vi "Cascade State.vi"(6 "First Iteration?":bool, 10 "Positions":T3, 11 "Cascade Motors":T1) -> (3 "Is Finished?":bool=TRUE)   [LabVIEW 2023]
uses:
  <vilib>/REV Custom Controls/Spark Output Control Type.ctl
  <vilib>/REVLibDriver/REVLibDriver.lvlib
  <resource>/objmgr/REVSpark.rc
  <vilib>/MRC/MrcLib.lvlib
  <vilib>/REV Custom Controls/SPARK Closed Loop Slot.ctl
  Cascade Positions.ctl
  <vilib>/REV Custom Controls/REVSparkRefnum.ctl
panel:
  in  "Cheat Factor":dbl=10.0
  out "Velocity":T2(graph)
  in  "dP":dbl
  out "Distance":dbl=-0.5875421712011715
  in  "Velocity Max":dbl=9000.0
  in  "Acceleration Max":dbl=9000.0
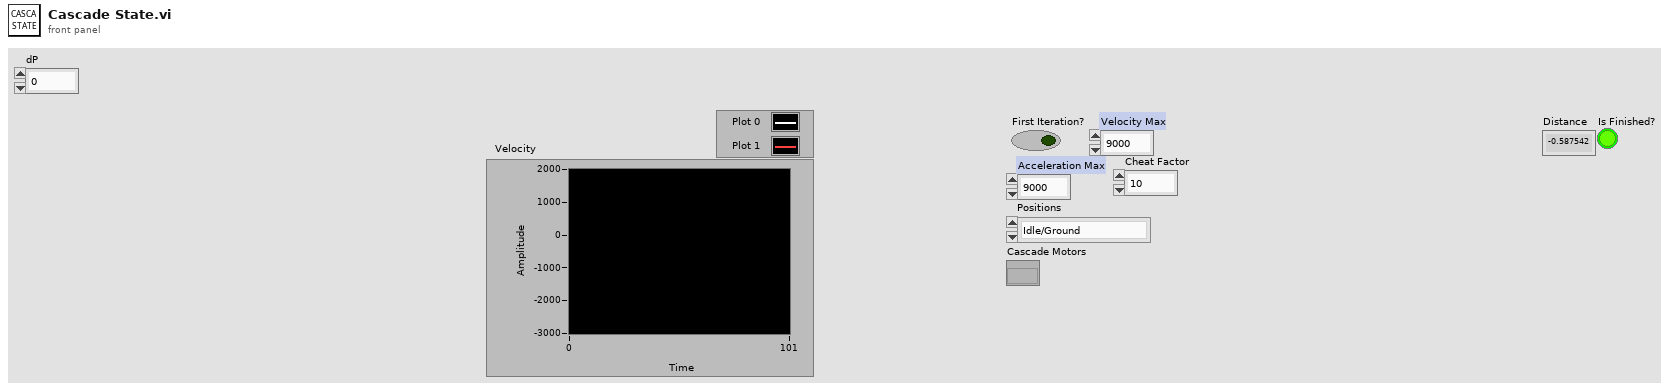
[diagram p1: front panel]
types:
  T1 = typedef "REVLibDriver.lvlib/REVSparkRefnum.ctl" = refnum<k20>
  T2 = cluster{"Numeric":dbl, "EncoderVelocityValue":sgl}
  T3 = typedef "Cascade Positions.ctl" = enum16{"Idle/Ground", "Raised L1", "L2", "L2 Tip", "L3", "L3 Tip", "Feeder", "\"Default\""}
  T4 = cluster{"Array":cluster{"Preset Name":T3, "Cascade Pos":dbl}[]}
  T5 = typedef "REVLibDriver.lvlib/Spark Output Control Type.ctl" = enum16{"Percent VBus", "Velocity", "Voltage", "Position", "Current", "MAXMotion Position", "MAXMotion Velocity"}
  T6 = typedef "SPARK Closed Loop Slot.ctl" = u16
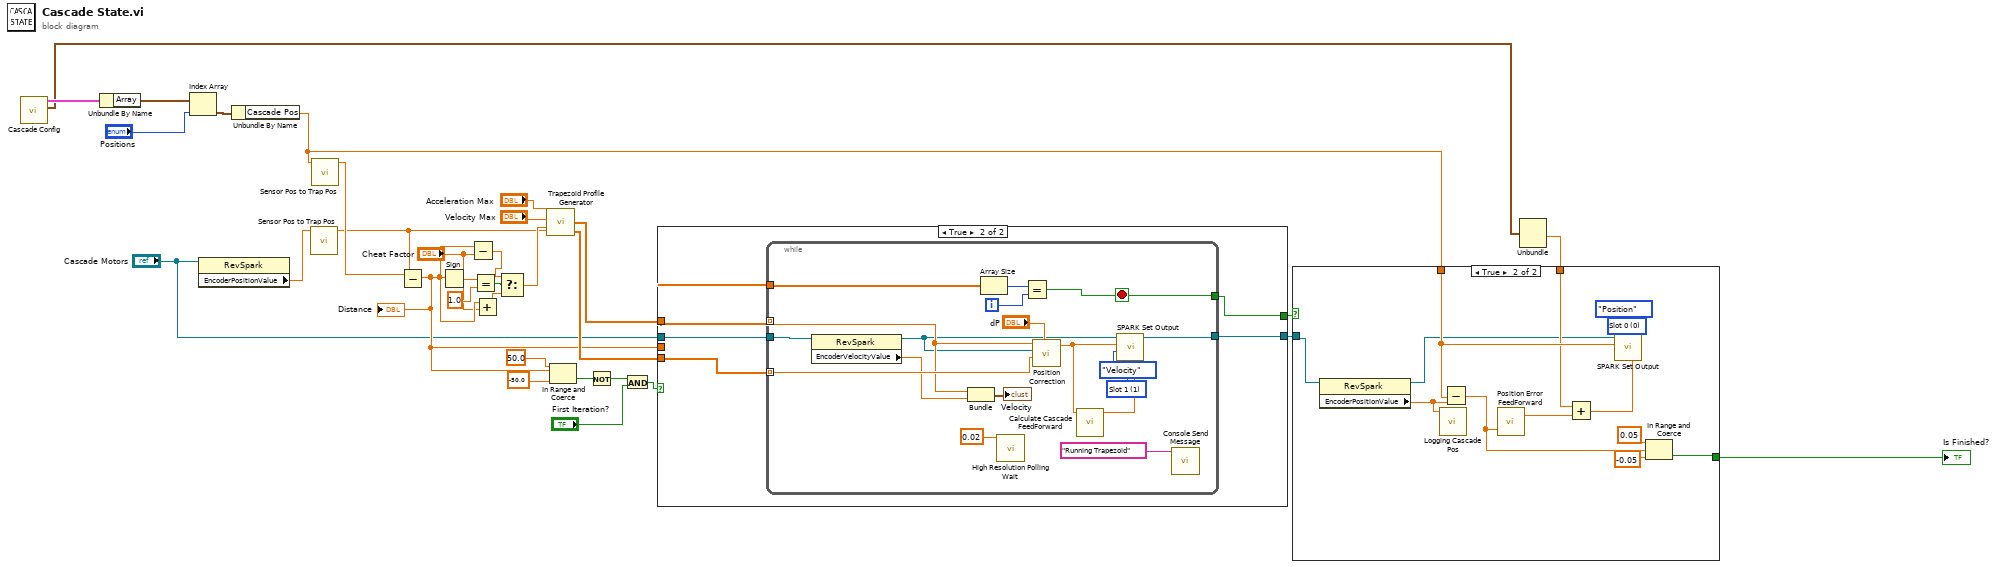
[diagram p0: block diagram]
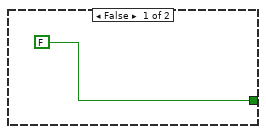
[diagram p2: hidden frame]
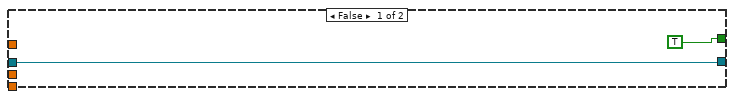
[diagram p3: hidden frame]
diagram:
  n1 = call "Cascade Config.vi"() -> ("FeedForward Constants Out"=w16:cluster{"kA":dbl, "kS":dbl, "kG":dbl, "kV":dbl}, "Cascade Setpoints Config Out (Sensor Positions)"=w32:T4)  [unwired: 10 in]
  n2 = Unbundle By Name(w32) -> ("Array"=w31:cluster{"Preset Name":T3, "Cascade Pos":dbl}[])
  n3 = Index Array(array=w31, index="Positions") -> (element=w30:cluster{"Preset Name":T3, "Cascade Pos":dbl})
  n4 = property class="RevSpark"(reference="Cascade Motors") -> ("EncoderPositionValue"=w23:sgl)  [unwired: 1 in, 2 out]
  n5 = Unbundle By Name(w30) -> ("Cascade Pos"=w25:dbl)
  n6 = call "Sensor Pos to Trap Pos.vi"("Sensor Pos"=w23) -> ("Trapezoid Pos"=w2:dbl)  [unwired: 10 in]
  n7 = call "Sensor Pos to Trap Pos.vi"("Sensor Pos"=w25) -> ("Trapezoid Pos"=w24:dbl)  [unwired: 10 in]
  n8 = Subtract(x=w24, y=w2) -> (x-y=w8:dbl)
  "Distance" <- w8
  n9 = Sign(1:w8) -> (0:w13:dbl)
  n10 = Subtract(x=w8, y="Cheat Factor") -> (x-y=w10:dbl)
  n11 = Equal?(x=w13, y=1.0 ("x")) -> (x = y?=w11:bool)
  n12 = Add(x=w8, y="Cheat Factor") -> (x+y=w9:dbl)
  n13 = Select(t=w10, s=w11, f=w9) -> (s? t:f=w6:dbl)
  n14 = call "Trapezoid Profile Generator.vi"("Starting Position"=w2, "Distance"=w6, "Velocity Max"="Velocity Max", "Acceleration Max"="Acceleration Max") -> ("Positions"=w22:dbl[], "Velocity values"=w27:dbl[])  [unwired: 5 in, 1 out]
  n15 = In Range and Coerce(upper limit=50.0, x=w8, lower limit=-50.0) -> (In Range?=w19:bool)  [unwired: 1 out]
  n16 = Not(x=w19) -> (.not. x?=w17:bool)
  n17 = And(x=w17, y="First Iteration?") -> (x .and. y?=w18:bool)
  n18 = case shown="True" w18 {
    tunnel: w27 -> [_ w39]
    tunnel: "Cascade Motors" -> [w33 w38]
    tunnel: [TRUE w37] -> w4
    tunnel: [w33 w36] -> w26
    tunnel: w22 -> [_ w35]
    tunnel: w8 -> [_ _]
    frame False {
    }
    frame True {
      n19 = while {
        tunnel: w39 -> [w47] mode=indexing
        tunnel: w38 -> [w46]
        tunnel: w39 -> [w56]
        tunnel: [w48] -> w37
        tunnel: [w53] -> w36
        tunnel: w35 -> [w52] mode=indexing
        i -> [w57]
        stop <- w48 stop-if-true
        w40 = T6 1 items=["Slot 0", "Slot 1", "Slot 2", "Slot 3"] ("Closed Loop Slot")
        n20 = property class="RevSpark"(reference=w46) -> (reference out=w42:T1, "EncoderVelocityValue"=w45:sgl)  [unwired: 1 in, 1 out]
        n21 = Bundle("Numeric"=w47, "EncoderVelocityValue"=w45) -> (→"Velocity":T2)  [unwired: 1 in]
        n22 = Array Size(array=w56) -> (size(s)=w55:i32)
        n23 = call <vilib>:"High Resolution Polling Wait.vi"("seconds to wait"=0.02) -> ()  [unwired: 10 in, 1 out]
        n24 = Equal?(x=w55, y=w57) -> (x = y?=w48:bool)
        n25 = call "Position Correction.vi"("dP"="dP", "Pos In"=w52, "RevSpark Session"=w42, "Velocity In"=w47) -> ("Velocity Out"=w51:dbl)  [unwired: 7 in]
        n26 = call "Calculate Cascade FeedForward.vi"("Setpoint"=w51) -> ("Arbitrary Feedforward"=w43:dbl)  [unwired: 10 in]
        n27 = call <vilib>:"SPARK Set Output.vi"("Arbitrary Feed Forward (0)"=w43, "Closed Loop Slot"=w40, "Control Mode"=Spark_Output_Control_Type."Velocity", "Setpoint"=w51, "Spark refnum"=w42) -> ("Spark refnum"=w53:T1)  [unwired: 5 in, 1 out]
        n28 = call <vilib>:"Console Send Message.vi"("Message"="Running Trapezoid") -> ()  [unwired: 14 in, 1 out]
      }
    }
  }
  n29 = Unbundle(w16) -> ("kG"=w15:dbl)  [unwired: 3 out]
  n30 = case shown="True" w4 {
    tunnel: w25 -> [_ w71]
    tunnel: w26 -> [_ w61]
    tunnel: [FALSE w69] -> w14
    tunnel: w15 -> [_ w70]
    frame False {
    }
    frame True {
      w59 = T6 0 items=["Slot 0", "Slot 1", "Slot 2", "Slot 3"] ("Closed Loop Slot")
      n31 = property class="RevSpark"(reference=w61) -> (reference out=w60:T1, "EncoderPositionValue"=w66:sgl)  [unwired: 1 in, 1 out]
      n32 = call "Logging Cascade Pos.vi"("Sensor Position"=w66) -> ()  [unwired: 11 in]
      n33 = Subtract(x=w66, y=w71) -> (x-y=w64:dbl)
      n34 = call "Position Error FeedForward.vi"("Position Error"=w64) -> (7:w63:dbl)  [unwired: 10 in]
      n35 = Add(x=w70, y=w63) -> (x+y=w65:dbl)
      n36 = call <vilib>:"SPARK Set Output.vi"("Arbitrary Feed Forward (0)"=w65, "Closed Loop Slot"=w59, "Control Mode"=Spark_Output_Control_Type."Position", "Setpoint"=w71, "Spark refnum"=w60) -> ()  [unwired: 5 in, 2 out]
      n37 = In Range and Coerce(upper limit=0.05, x=w64, lower limit=-0.05) -> (In Range?=w69:bool)  [unwired: 1 out]
    }
  }
  "Is Finished?" <- w14
